vi "Write destination.vi"(8 "error in (no error)":errorcluster, 10 "ZM-PC-DESTINATION":T1, 11 "ZM-PC-package in":refnum<class "ZM-PC-package.lvclass">) -> (0 "error out":errorcluster, 3 "ZM-PC-package out":refnum<class "ZM-PC-package.lvclass">)   [LabVIEW 2020, in "ZM-PC-packages.lvlib" / "ZM-PC-package.lvclass"]
doc: "Writes one field of this class's private data. Generated by lvai_create_accessors from the class private data control."
uses:
  ZM-PC-package.lvclass
  ZM-PC-package.lvclass/ZM-PC-package.ctl
  ZM-PC-DESTINATION.ctl
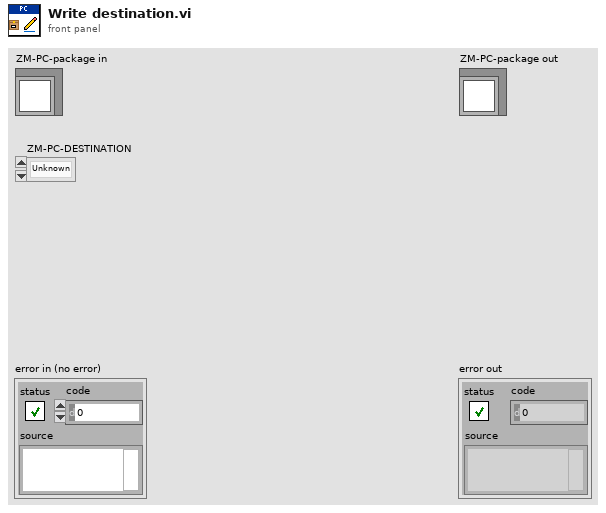
[diagram p1: front panel]
types:
  T1 = typedef "ZM-PC-packages.lvlib/ZM-PC-package.lvclass/ZM-PC-DESTINATION.ctl" = enum16{"Unknown", "Root", "Hardware", "Communication"}
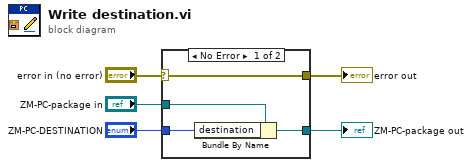
[diagram p0: block diagram]
diagram:
  n1 = case shown="No Error" "error in (no error)" {
    selector: "error in (no error)" -> [w9 w10]
    tunnel: [w9 w10] -> w4
    tunnel: [w7 w11] -> w2
    tunnel: "ZM-PC-package in" -> [w8 w11]
    tunnel: "ZM-PC-DESTINATION" -> [w6 _]
    frame No Error {
      n2 = Bundle By Name(cluster=w8, "destination"=w6) -> (w7:refnum<class "ZM-PC-package.lvclass">)
    }
    frame Error {
    }
  }
  "error out" <- w4
  "ZM-PC-package out" <- w2
